vi "test tools list descriptions defaults ranges.vi"(8 "error in (no error)":errorcluster) -> (0 "error out":errorcluster, 3 "body":string)   [LabVIEW 2020, in "MCP Server tests.lvlib"]
doc: "tools/list must describe each input completely enough for a model: the descriptions of cluster elements at any depth (also inside an array of clusters), integer ranges from the representation, the data entry limits of numeric controls, the unit of a numeric with a unit, and the default of inputs that are not required. fake_tool_schema_details is found by its MCP name: level (U8, default 7) has minimum 0, maximum 255 and default 7; setpoint (DBL, data entry limits 0 to 100, coerced, default 25) has minimum 0, maximum 100 and default 25; voltage (unit V) has the description \"Supply voltage. Unit: V.\"; the element descriptions of config arrive under properties, also inside the array of clusters, and gain, which has none, has no description; count is required, so it has no default, and has the I32 range; mode (enum) has the default \"fast\". The integer items of matrix in fake_tool_schema_shapes have the I32 minimum. The request is sent with the LabVIEW HTTP Client directly."
uses:
  MCP Server tests.lvlib
  4f187fbe-bcda-47a0-bee9-e9e270e05a99.vi
  db1147a5-3762-472d-a5ee-aa4910886604.vi
  <vilib>/JDP Science/JSONtext/Next JSON Value.vi
  <vilib>/JDP Science/JSONtext/String Subset.vi
  <vilib>/JDP Science/JSONtext/Parsing/Advance past next JSON Value (inlined COPY).vi
  <vilib>/JDP Science/JSONtext/Parsing/Advance past whitespace.vi
  <vilib>/JDP Science/JSONtext/Parsing/Advance past String.vi
  <vilib>/JDP Science/JSONtext/Parsing/Advance past Number.vi
  <vilib>/JDP Science/JSONtext/Parsing/Advance past Line Ending.vi
  <vilib>/JDP Science/JSONtext/Parsing/Parse Full Path or Item Name.vi
  <vilib>/JDP Science/JSONtext/Parsing/Advance past Array.vi
  <vilib>/JDP Science/JSONtext/Parsing/Advance past Object.vi
  <vilib>/JDP Science/JSONtext/support/Error Cluster From Code.vi
  <vilib>/JDP Science/JSONtext/Offset/Find Item Locations by Path.vi
  <vilib>/JDP Science/JSONtext/JSON text to Variant.vi
  <vilib>/JDP Science/JSONtext/LVClass Serializer/JSONtext LVClass Serializer.lvclass
  <vilib>/addons/_JKI Toolkits/Caraya/classes/Test/Test.lvclass
  <vilib>/JDP Science/JSONtext/JSONtext.lvlib
  <vilib>/addons/_JKI Toolkits/Caraya/classes/Assert/Assert.lvclass
panel:
  out "lookup error":errorcluster
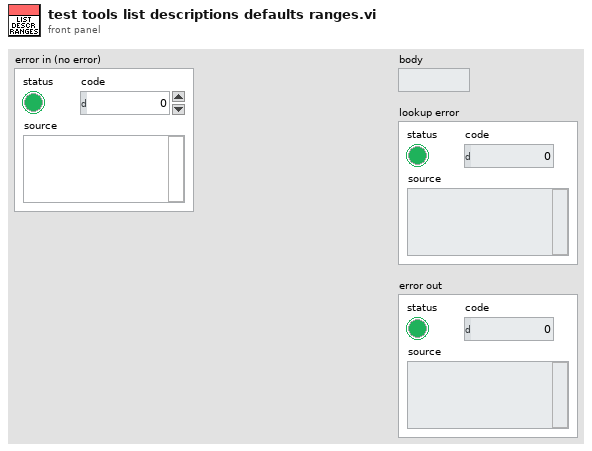
[diagram p1: front panel]
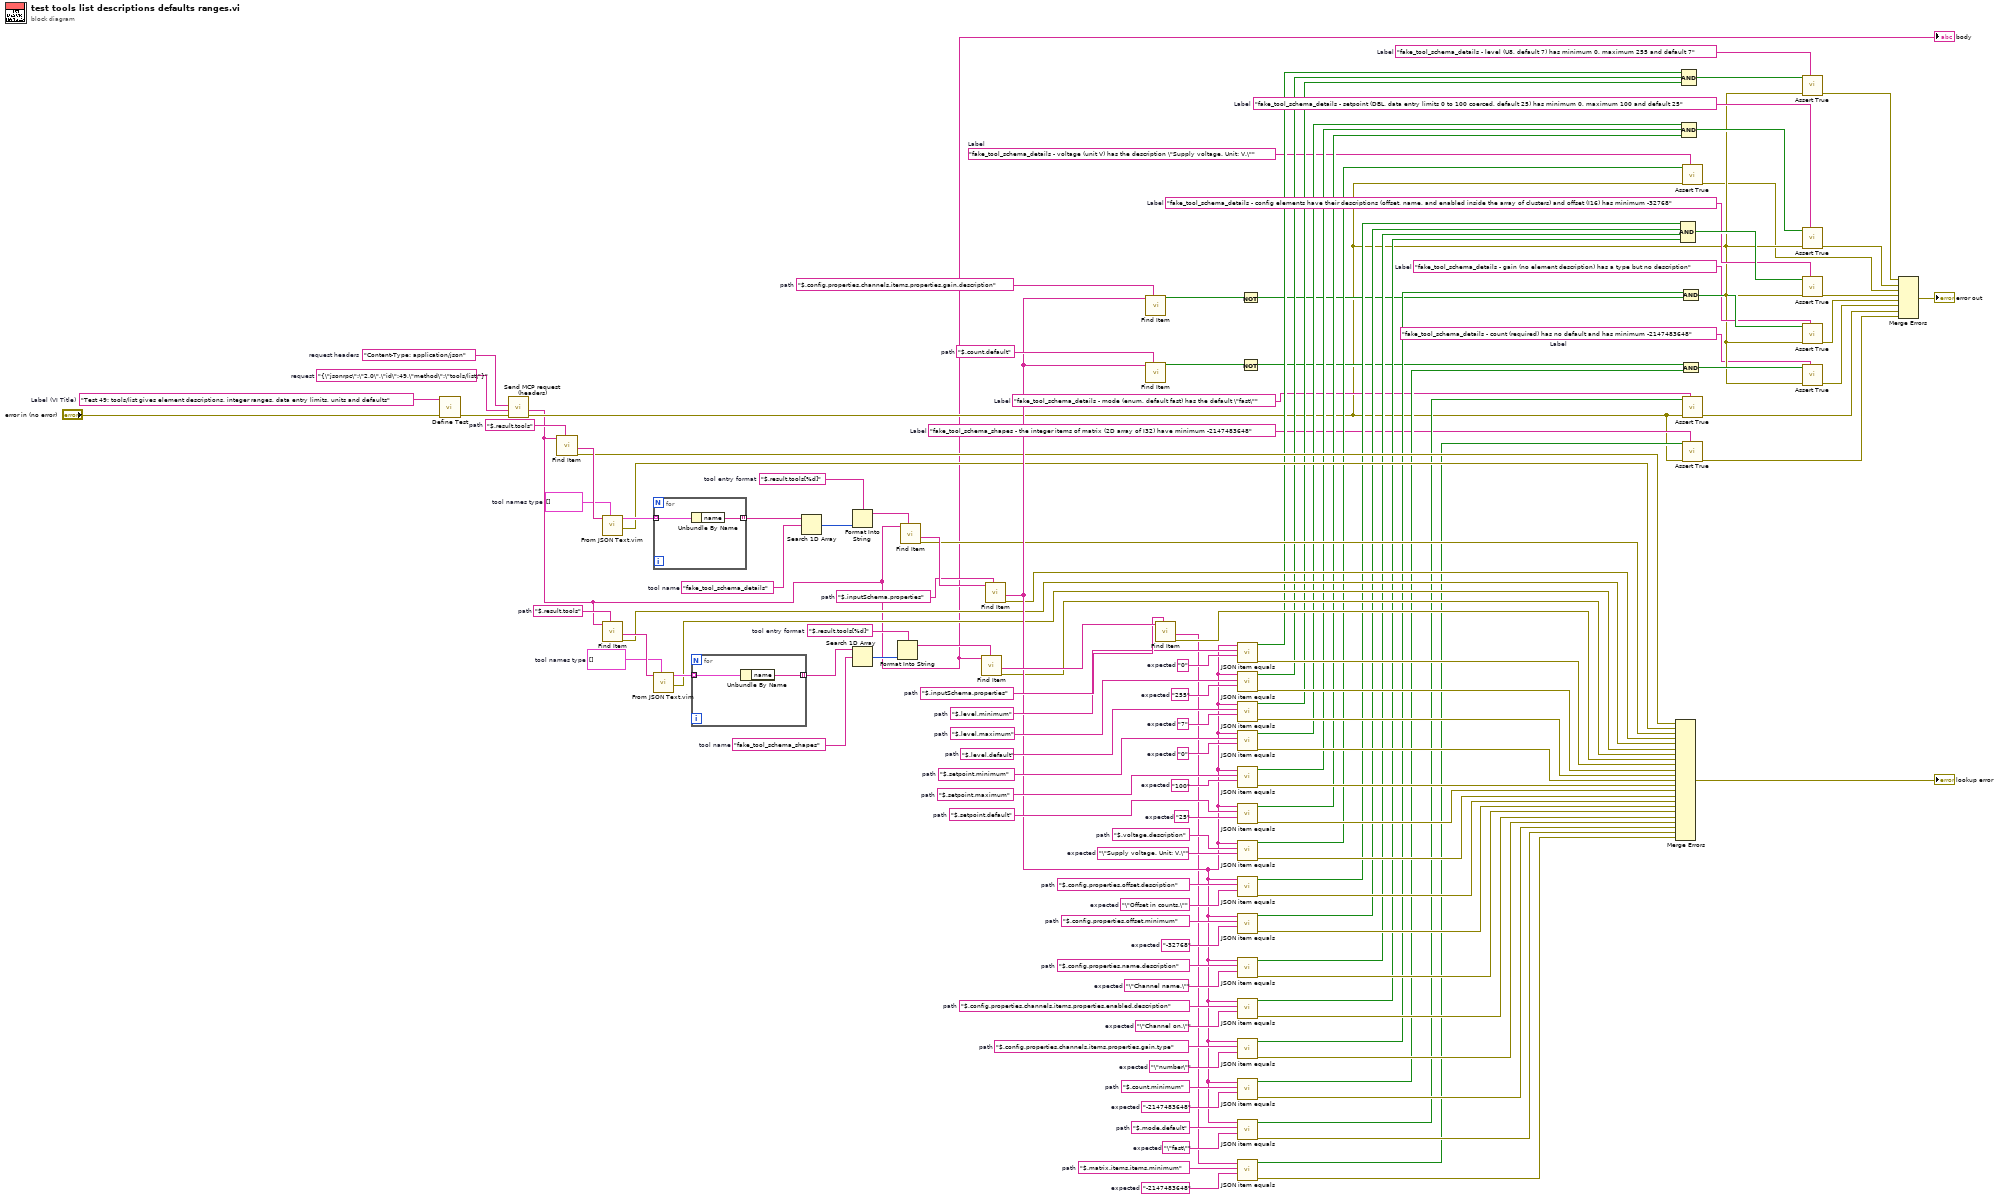
[diagram p0: block diagram]
diagram:
  w126 = "Content-Type: application/json"  # request headers
  w23 = "fake_tool_schema_shapes - the integer items of matrix (2D array of I32) have minimum -2147483648"  # Label
  w25 = "fake_tool_schema_details - mode (enum, default fast) has the default \"fast\""  # Label
  w12 = "fake_tool_schema_details - count (required) has no default and has minimum -2147483648"  # Label
  w15 = "fake_tool_schema_details - gain (no element description) has a type but no description"  # Label
  w17 = "fake_tool_schema_details - config elements have their descriptions (offset, name, and enabled inside the array of clusters) and offset (I16) has minimum -32768"  # Label
  w35 = "fake_tool_schema_details - voltage (unit V) has the description \"Supply voltage. Unit: V.\""  # Label
  w19 = "fake_tool_schema_details - setpoint (DBL, data entry limits 0 to 100 coerced, default 25) has minimum 0, maximum 100 and default 25"  # Label
  w21 = "fake_tool_schema_details - level (U8, default 7) has minimum 0, maximum 255 and default 7"  # Label
  w44 = "-2147483648"  # expected
  w45 = "$.matrix.items.items.minimum"  # path
  w69 = "\"fast\""  # expected
  w70 = "$.mode.default"  # path
  w72 = "-2147483648"  # expected
  w73 = "$.count.minimum"  # path
  w100 = "$.count.default"  # path
  w101 = "$.config.properties.channels.items.properties.gain.description"  # path
  w76 = "\"number\""  # expected
  w77 = "$.config.properties.channels.items.properties.gain.type"  # path
  w78 = "\"Channel on.\""  # expected
  w79 = "$.config.properties.channels.items.properties.enabled.description"  # path
  w80 = "\"Channel name.\""  # expected
  w81 = "$.config.properties.name.description"  # path
  w82 = "-32768"  # expected
  w83 = "$.config.properties.offset.minimum"  # path
  w84 = "\"Offset in counts.\""  # expected
  w85 = "$.config.properties.offset.description"  # path
  w86 = "\"Supply voltage. Unit: V.\""  # expected
  w87 = "$.voltage.description"  # path
  w88 = "25"  # expected
  w89 = "$.setpoint.default"  # path
  w90 = "100"  # expected
  w91 = "$.setpoint.maximum"  # path
  w92 = "0"  # expected
  w93 = "$.setpoint.minimum"  # path
  w94 = "7"  # expected
  w95 = "$.level.default"  # path
  w96 = "255"  # expected
  w97 = "$.level.maximum"  # path
  w98 = "0"  # expected
  w99 = "$.level.minimum"  # path
  w102 = "$.inputSchema.properties"  # path
  w108 = "$.result.tools[%d]"  # tool entry format
  w112 = "fake_tool_schema_shapes"  # tool name
  w118 = cluster{"name":string}[] []  # tool names type
  w122 = "$.result.tools"  # path
  w104 = "$.inputSchema.properties"  # path
  w110 = "$.result.tools[%d]"  # tool entry format
  w114 = "fake_tool_schema_details"  # tool name
  w120 = cluster{"name":string}[] []  # tool names type
  w123 = "$.result.tools"  # path
  w125 = "{\"jsonrpc\":\"2.0\",\"id\":49,\"method\":\"tools/list\"}"  # request
  w128 = "Test 49: tools/list gives element descriptions, integer ranges, data entry limits, units and defaults"  # Label (VI Title)
  n1 = call <vilib>:"Define Test.vi"("error in (no error)"="error in (no error)", "Label (VI Title)"=w128) -> ("error out"=w124:errorcluster)  [unwired: 8 in, 1 out]
  n2 = call "Send MCP request (headers).vi"("error in (no error)"=w124, "request"=w125, "request headers"=w126) -> ("error out"=w13:errorcluster, "response"=w3:string)  [unwired: 5 in, 2 out]
  "body" <- w3
  n3 = call <vilib>:"Find Item.vi"("$Path or Item Name"=w123, "JSON"=w3) -> ("error out"=w68:errorcluster, "<JSON>"=w121:string)  [unwired: 6 in, 2 out]
  n4 = call "From JSON Text.vim"("Data Type and Default Value"=w120, "JSON"=w121) -> ("error out"=w67:errorcluster, "Data out"=w117:cluster{"name":string}[])  [unwired: 8 in]
  n5 = call <vilib>:"Find Item.vi"("$Path or Item Name"=w122, "JSON"=w3) -> ("error out"=w64:errorcluster, "<JSON>"=w119:string)  [unwired: 6 in, 2 out]
  n6 = for {
    tunnel: w117 -> [w130] mode=indexing
    tunnel: [w129] -> w115 mode=indexing
    n7 = Unbundle By Name(w130) -> ("name"=w129:string)
  }
  n8 = call "From JSON Text.vim"("Data Type and Default Value"=w118, "JSON"=w119) -> ("error out"=w63:errorcluster, "Data out"=w116:cluster{"name":string}[])  [unwired: 8 in]
  n9 = for {
    tunnel: w116 -> [w132] mode=indexing
    tunnel: [w131] -> w113 mode=indexing
    n10 = Unbundle By Name(w132) -> ("name"=w131:string)
  }
  n11 = Search 1D Array(1D array=w115, element=w114) -> (index of element=w111:i32)  [unwired: 1 in]
  n12 = Format Into String(format string=w110, w111) -> (resulting string=w107:string)  [unwired: 2 in, 1 out]
  n13 = Search 1D Array(1D array=w113, element=w112) -> (index of element=w109:i32)  [unwired: 1 in]
  n14 = Format Into String(format string=w108, w109) -> (resulting string=w106:string)  [unwired: 2 in, 1 out]
  n15 = call <vilib>:"Find Item.vi"("$Path or Item Name"=w107, "JSON"=w3) -> ("error out"=w66:errorcluster, "<JSON>"=w105:string)  [unwired: 6 in, 2 out]
  n16 = call <vilib>:"Find Item.vi"("$Path or Item Name"=w106, "JSON"=w3) -> ("error out"=w62:errorcluster, "<JSON>"=w103:string)  [unwired: 6 in, 2 out]
  n17 = call <vilib>:"Find Item.vi"("$Path or Item Name"=w104, "JSON"=w105) -> ("error out"=w65:errorcluster, "<JSON>"=w71:string)  [unwired: 6 in, 2 out]
  n18 = call <vilib>:"Find Item.vi"("$Path or Item Name"=w101, "JSON"=w71) -> ("Found"=w75:bool)  [unwired: 6 in, 3 out]
  n19 = call <vilib>:"Find Item.vi"("$Path or Item Name"=w100, "JSON"=w71) -> ("Found"=w74:bool)  [unwired: 6 in, 3 out]
  n20 = call <vilib>:"Find Item.vi"("$Path or Item Name"=w102, "JSON"=w103) -> ("error out"=w61:errorcluster, "<JSON>"=w46:string)  [unwired: 6 in, 2 out]
  n21 = call "JSON item equals.vi"("expected"=w98, "path"=w99, "JSON"=w71) -> ("error out"=w60:errorcluster, "equal?"=w42:bool)  [unwired: 6 in, 1 out]
  n22 = call "JSON item equals.vi"("expected"=w96, "path"=w97, "JSON"=w71) -> ("error out"=w59:errorcluster, "equal?"=w41:bool)  [unwired: 6 in, 1 out]
  n23 = call "JSON item equals.vi"("expected"=w94, "path"=w95, "JSON"=w71) -> ("error out"=w58:errorcluster, "equal?"=w40:bool)  [unwired: 6 in, 1 out]
  n24 = call "JSON item equals.vi"("expected"=w92, "path"=w93, "JSON"=w71) -> ("error out"=w57:errorcluster, "equal?"=w39:bool)  [unwired: 6 in, 1 out]
  n25 = call "JSON item equals.vi"("expected"=w90, "path"=w91, "JSON"=w71) -> ("error out"=w56:errorcluster, "equal?"=w38:bool)  [unwired: 6 in, 1 out]
  n26 = call "JSON item equals.vi"("expected"=w88, "path"=w89, "JSON"=w71) -> ("error out"=w55:errorcluster, "equal?"=w37:bool)  [unwired: 6 in, 1 out]
  n27 = call "JSON item equals.vi"("expected"=w86, "path"=w87, "JSON"=w71) -> ("error out"=w54:errorcluster, "equal?"=w36:bool)  [unwired: 6 in, 1 out]
  n28 = call "JSON item equals.vi"("expected"=w84, "path"=w85, "JSON"=w71) -> ("error out"=w53:errorcluster, "equal?"=w34:bool)  [unwired: 6 in, 1 out]
  n29 = call "JSON item equals.vi"("expected"=w82, "path"=w83, "JSON"=w71) -> ("error out"=w52:errorcluster, "equal?"=w33:bool)  [unwired: 6 in, 1 out]
  n30 = call "JSON item equals.vi"("expected"=w80, "path"=w81, "JSON"=w71) -> ("error out"=w51:errorcluster, "equal?"=w32:bool)  [unwired: 6 in, 1 out]
  n31 = call "JSON item equals.vi"("expected"=w78, "path"=w79, "JSON"=w71) -> ("error out"=w50:errorcluster, "equal?"=w31:bool)  [unwired: 6 in, 1 out]
  n32 = call "JSON item equals.vi"("expected"=w76, "path"=w77, "JSON"=w71) -> ("error out"=w49:errorcluster, "equal?"=w30:bool)  [unwired: 6 in, 1 out]
  n33 = call "JSON item equals.vi"("expected"=w72, "path"=w73, "JSON"=w71) -> ("error out"=w48:errorcluster, "equal?"=w27:bool)  [unwired: 6 in, 1 out]
  n34 = call "JSON item equals.vi"("expected"=w69, "path"=w70, "JSON"=w71) -> ("error out"=w47:errorcluster, "equal?"=w26:bool)  [unwired: 6 in, 1 out]
  n35 = call "JSON item equals.vi"("expected"=w44, "path"=w45, "JSON"=w46) -> ("error out"=w43:errorcluster, "equal?"=w24:bool)  [unwired: 6 in, 1 out]
  n36 = Not(x=w75) -> (.not. x?=w29:bool)
  n37 = Not(x=w74) -> (.not. x?=w28:bool)
  n38 = Merge Errors(w68, w67, w66, w65, w64, w63, w62, w61, w60, w59, w58, w57, w56, w55, w54, w53, w52, w51, w50, w49, w48, w47, w43) -> (→"lookup error":errorcluster)
  n39 = Compound Arithmetic op=AND(w34, w33, w32, w31) -> (w18:bool)
  n40 = Compound Arithmetic op=AND(w42, w41, w40) -> (w22:bool)
  n41 = Compound Arithmetic op=AND(w39, w38, w37) -> (w20:bool)
  n42 = call <vilib>:"Assert True.vi"("Label"=w35, "error in (no error)"=w13, "True?"=w36) -> ("error out"=w9:errorcluster)  [unwired: 7 in, 1 out]
  n43 = call <vilib>:"Assert True.vi"("Label"=w25, "error in (no error)"=w13, "True?"=w26) -> ("error out"=w5:errorcluster)  [unwired: 7 in, 1 out]
  n44 = call <vilib>:"Assert True.vi"("Label"=w23, "error in (no error)"=w13, "True?"=w24) -> ("error out"=w4:errorcluster)  [unwired: 7 in, 1 out]
  n45 = Compound Arithmetic op=AND(w30, w29) -> (w16:bool)
  n46 = Compound Arithmetic op=AND(w28, w27) -> (w14:bool)
  n47 = call <vilib>:"Assert True.vi"("Label"=w21, "error in (no error)"=w13, "True?"=w22) -> ("error out"=w11:errorcluster)  [unwired: 7 in, 1 out]
  n48 = call <vilib>:"Assert True.vi"("Label"=w19, "error in (no error)"=w13, "True?"=w20) -> ("error out"=w10:errorcluster)  [unwired: 7 in, 1 out]
  n49 = call <vilib>:"Assert True.vi"("Label"=w17, "error in (no error)"=w13, "True?"=w18) -> ("error out"=w8:errorcluster)  [unwired: 7 in, 1 out]
  n50 = call <vilib>:"Assert True.vi"("Label"=w15, "error in (no error)"=w13, "True?"=w16) -> ("error out"=w7:errorcluster)  [unwired: 7 in, 1 out]
  n51 = call <vilib>:"Assert True.vi"("Label"=w12, "error in (no error)"=w13, "True?"=w14) -> ("error out"=w6:errorcluster)  [unwired: 7 in, 1 out]
  n52 = Merge Errors(w11, w10, w9, w8, w7, w6, w5, w4) -> (→"error out":errorcluster)
